vi "Get Device List.vi"(8 "error in":errorcluster) -> (0 "error out":errorcluster, 3 "Device List":string[](array[string]))   [LabVIEW 2021, in "USB Relay Control.lvlib"]
uses:
  USB Relay Control.lvlib
  hid.dll
  cfgmgr32.dll
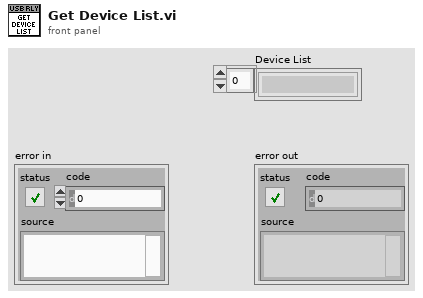
[diagram p1: front panel]
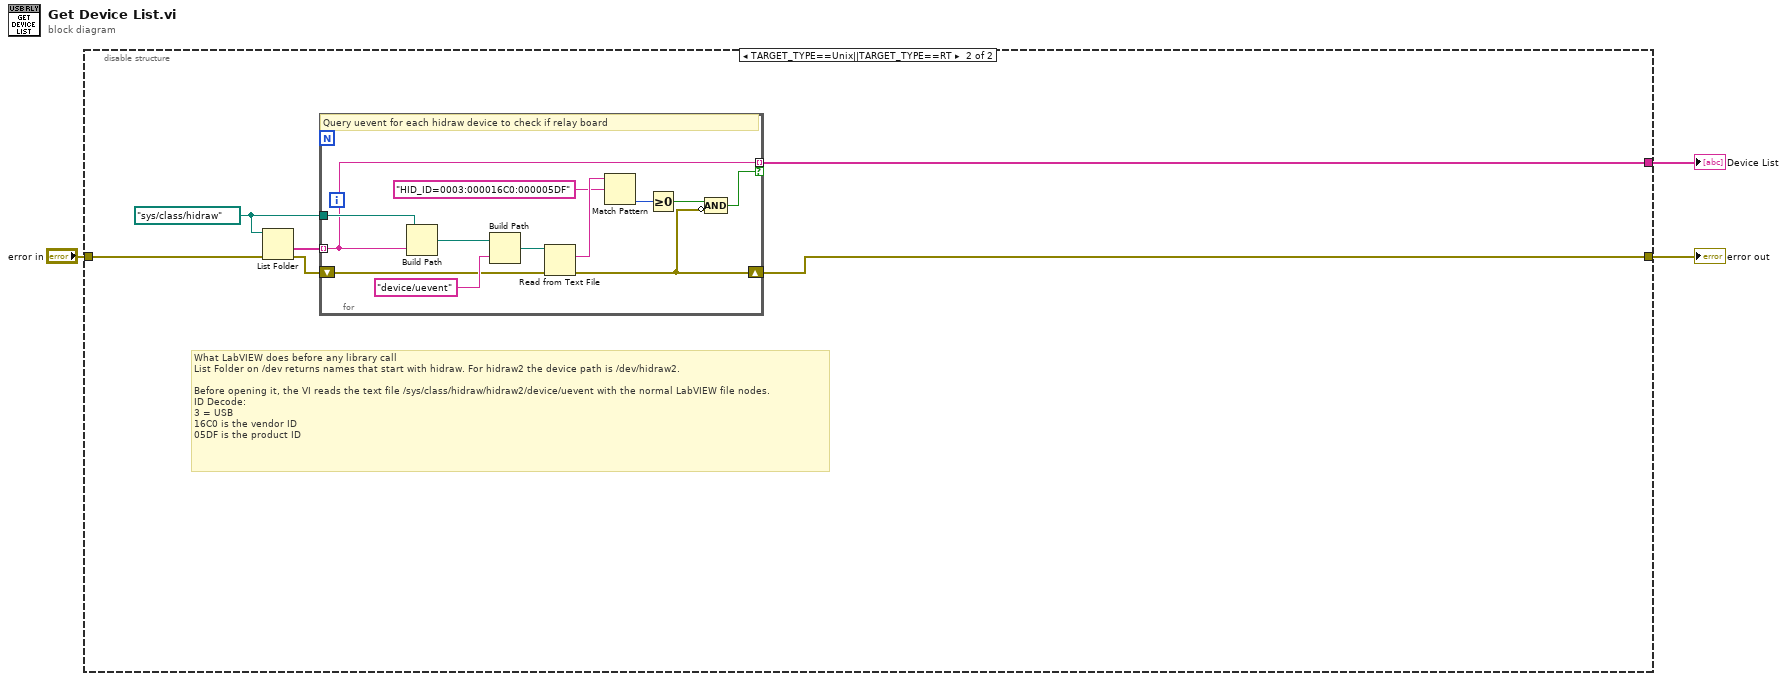
[diagram p0: block diagram]
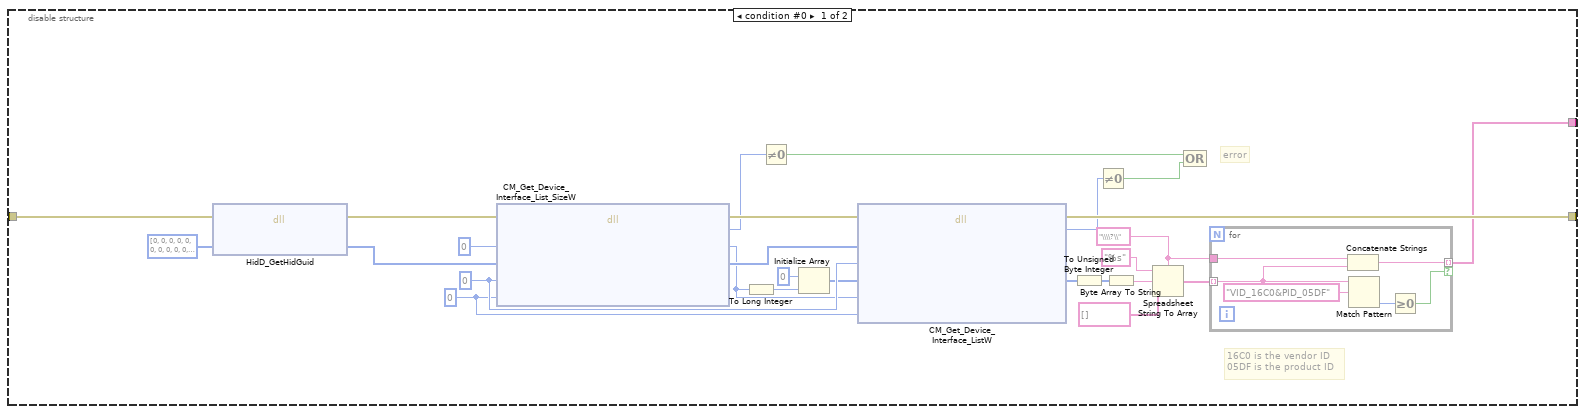
[diagram p2: hidden frame]
diagram:
  n1 = disable-structure shown="TARGET_TYPE==Unix||TARGET_TYPE==RT" {
    disable-tunnel: [w10 w39] -> w3
    disable-tunnel: "error in" -> [w28 w37]
    disable-tunnel: [w23 w36] -> w1
    frame condition #0 {
      w4 = "\\\\?\\" ("delimiter (Tab)")
      w17 = u32 0 ("ulFlags")
      w21 = u64 0 ("pDeviceID")
      # "error"
      # "16C0 is the vendor ID\n05DF is the product ID"
      n2 = dll-call lib="hid.dll" fn="HidD_GetHidGuid"(error in=w28, "GUID"=u8[] [0, 0, 0, 0, 0, 0, 0, 0, 0, 0, 0, 0, 0, 0, 0, 0]) -> (error out=w27:errorcluster, "GUID"=w25:u8[])  [unwired: 3 in, 1 out]
      n3 = dll-call lib="cfgmgr32.dll" fn="CM_Get_Device_Interface_List_SizeW"(error in=w27, "pulLen"=u32 0, "InterfaceClassGuid"=w25, "pDeviceID"=w21, "ulFlags"=w17) -> (error out=w24:errorcluster, "return type"=w9:u32, "pulLen"=w18:u32, "InterfaceClassGuid"=w22:u8[])  [unwired: 4 in, 1 out]
      n4 = To Long Integer(number=w18) -> (32bit integer=w5:i32)
      n5 = Not Equal To 0?(x=w9) -> (x != 0?=w6:bool)
      n6 = Initialize Array(u16 0 ("element"), w5) -> (w19:u16[])
      n7 = dll-call lib="cfgmgr32.dll" fn="CM_Get_Device_Interface_ListW"(error in=w24, "InterfaceClassGuid"=w22, "pDeviceID"=w21, "Buffer"=w19, "BufferLen"=w18, "ulFlags"=w17) -> (error out=w23:errorcluster, "return type"=w8:u32, "Buffer"=w16:u16[])  [unwired: 6 in, 1 out]
      n8 = To Unsigned Byte Integer(number=w16) -> (unsigned 8bit integer=w11:u8[])
      n9 = Not Equal To 0?(x=w8) -> (x != 0?=w7:bool)
      n10 = Byte Array To String(unsigned byte array=w11) -> (string=w12:string)
      n11 = Spreadsheet String To Array(delimiter (Tab)=w4, format string="%s", spreadsheet string=w12, array type (2D Dbl)=string[] []) -> (array=w13:string[])
      n12 = Compound Arithmetic op=OR(w6, w7) -> ()  [unwired: 1 out]
      n13 = for {
        tunnel: w13 -> [w32] mode=indexing
        tunnel: [w30] -> w10 mode=indexing if=w33
        tunnel: w4 -> [w31]
        n14 = Concatenate Strings(w31, w32) -> (w30:string)
        n15 = Match Pattern(string=w32, regular expression="VID_16C0&PID_05DF") -> (offset past match=w34:i32)  [unwired: 1 in, 3 out]
        n16 = Greater Or Equal To 0?(x=w34) -> (x >= 0?=w33:bool)
      }
    }
    frame condition #1 (active) {
      w40 = path "/sys/class/hidraw" ("path")
      # "What LabVIEW does before any library call\nList Folder on /dev returns names that start with hidraw. For hidraw2 the device path is /dev/hidraw2.\n\nBefore opening it, the VI reads the text file /sys/class/hidraw/hidraw2/device/uevent with the normal LabVIEW file nodes.\nID Decode:\n3 = USB\n16C0 is the vendor ID\n05DF is the product ID"
      n17 = List Folder(path=w40, error in=w37) -> (folder names=w41:string[], error out=w38:errorcluster)  [unwired: 2 in, 2 out]
      n18 = for {
        tunnel: w41 -> [w46] mode=indexing
        tunnel: w40 -> [w53]
        tunnel: [w46] -> w39 mode=indexing if=w44
        shift-right: [w43] -> w36
        shift-left: w38 -> [w42]
        # "Query uevent for each hidraw device to check if relay board"
        n19 = Build Path(base path=w53, name or relative path=w46) -> (appended path=w52:path)
        n20 = Build Path(base path=w52, name or relative path="device/uevent") -> (appended path=w50:path)
        n21 = Read from Text File(file (use dialog)=w50, error in=w42) -> (text=w49:string, error out=w43:errorcluster)  [unwired: 2 in, 2 out]
        n22 = Match Pattern(string=w49, regular expression="HID_ID=0003:000016C0:000005DF") -> (offset past match=w47:i32)  [unwired: 1 in, 3 out]
        n23 = Greater Or Equal To 0?(x=w47) -> (x >= 0?=w45:bool)
        n24 = Compound Arithmetic op=AND(w45, invert w43) -> (w44:bool)
      }
    }
  }
  "Device List" <- w3
  "error out" <- w1
